vi "avalanche.vi"() -> ()   [LabVIEW 2018]
panel:
  out "Collision":bool
  out "High Score":u32
  in  "Difficulty":dbl
  out "Key Down":bool
  out "Key Up":bool
  out "Height":i32
  out "Key Right":bool
  out "Key Left":bool
  out "Final Score":i32
  out "% Passed":dbl
  in  "stop":bool
  out "Current Score":i32
  out "XY Graph":cluster{dbl[], i32[]}(graph)
  out "Position":dbl
  out "error out":errorcluster
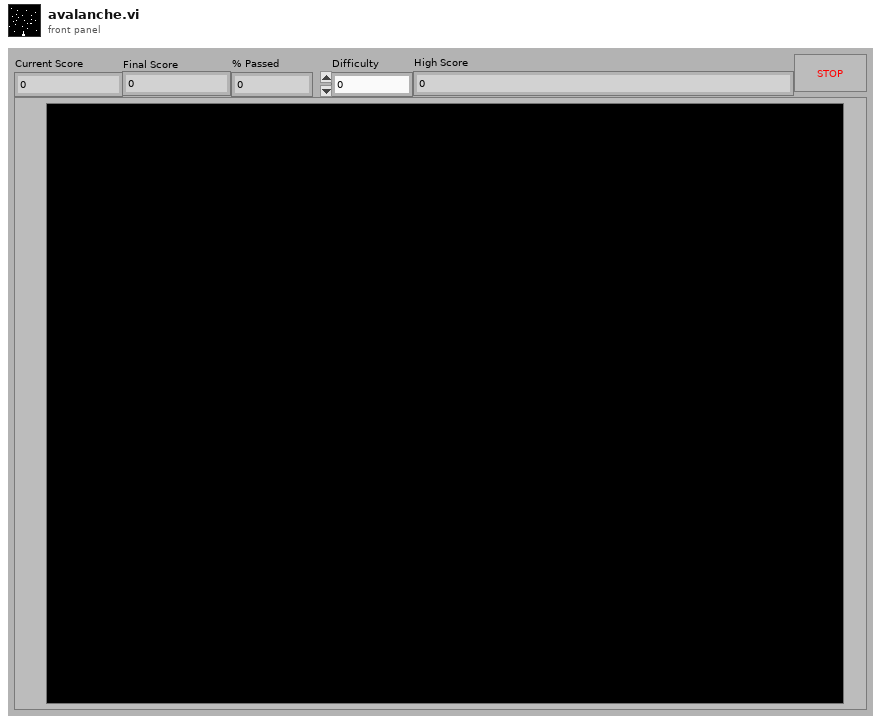
[diagram p1: front panel]
types:
  T1 = typedef "eventvkey.ctl" = enum16{"ASCII", "Enter", "Return", "Shift", "Ctrl", "Alt", "Cmd", "Opt", "Caps", "NumLock", "Clear", "Break", "Up", "Down", "Left", "Right", "Insert", "Delete", "Home", "End", "PageUp", "PageDown", "Escape", "Help", "Pause", "ScrollLock", "F1", "F2", "F3", "F4", "F5", "F6", "F7", "F8", "F9", "F10", "F11", "F12", "F13", "F14", "F15", "F16", "F17", "F18", "F19", "F20", "F21", "F22", "F23", "F24", "Play", "VolumeUp", "VolumeDown", "Mute", "Two Byte Char"}
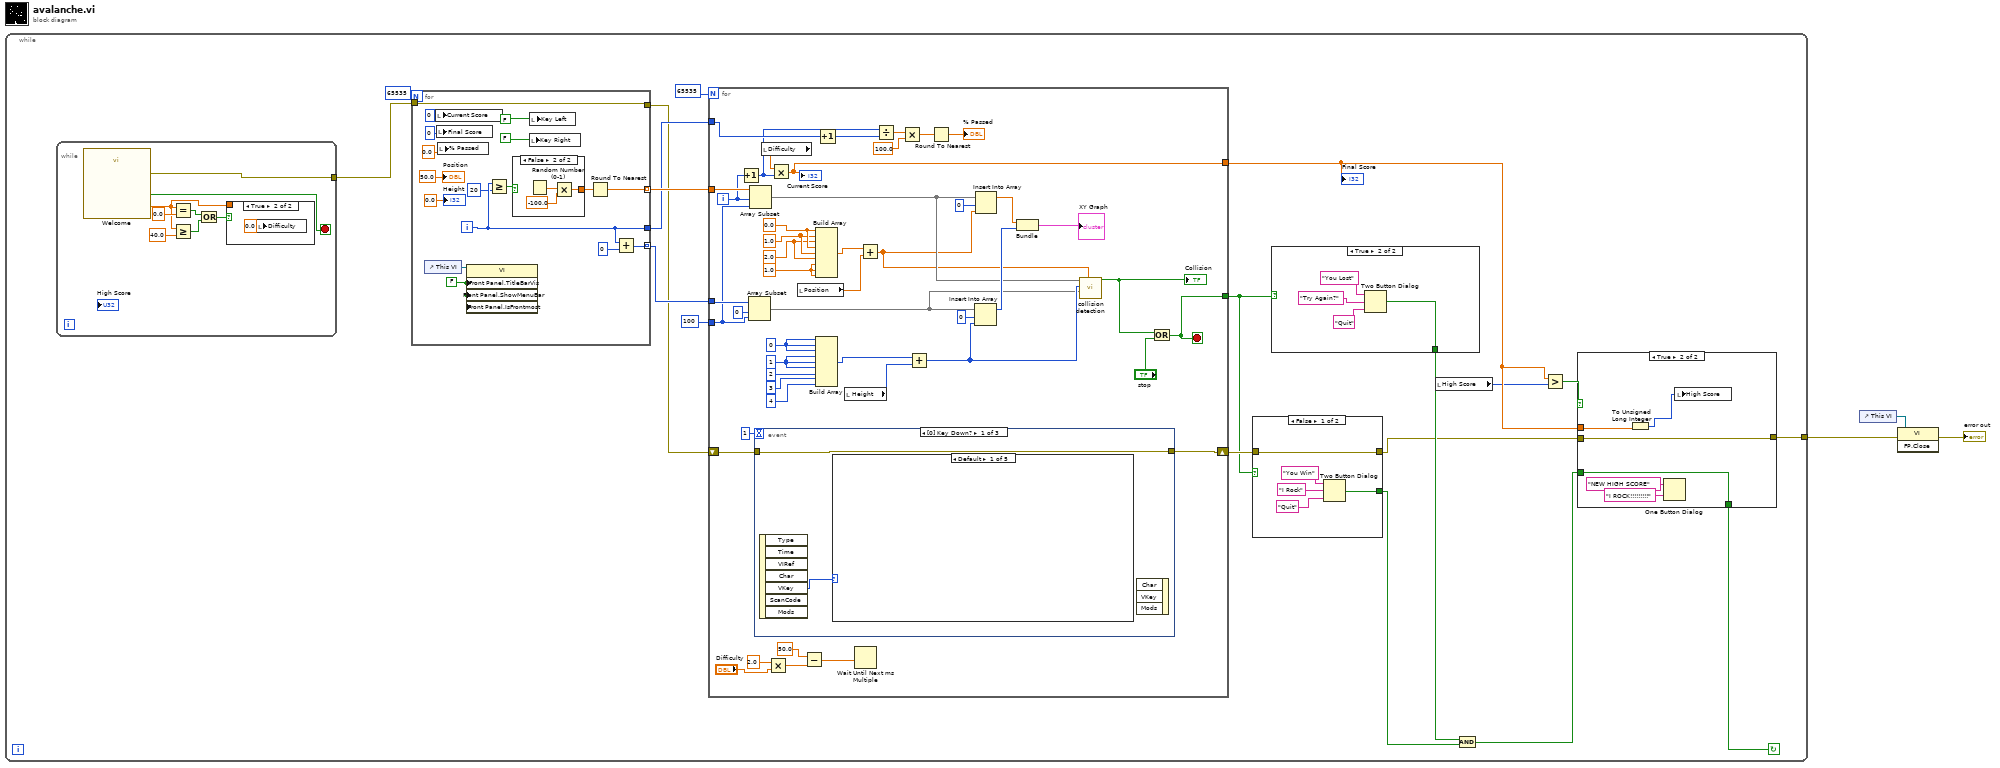
[diagram p0: block diagram]
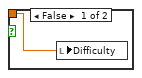
[diagram p3: hidden frame]
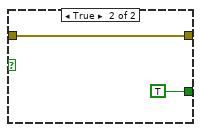
[diagram p4: hidden frame]
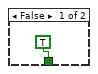
[diagram p5: hidden frame]
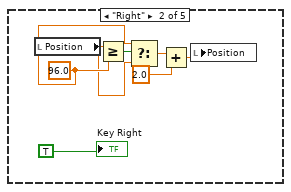
[diagram p6: hidden frame]
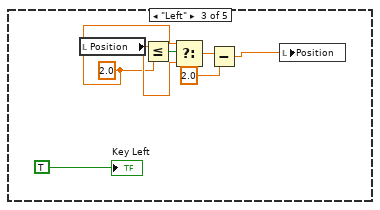
[diagram p7: hidden frame]
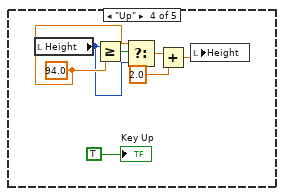
[diagram p8: hidden frame]
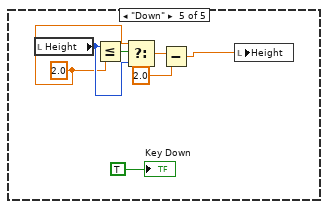
[diagram p9: hidden frame]
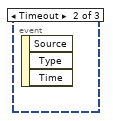
[diagram p10: hidden frame]
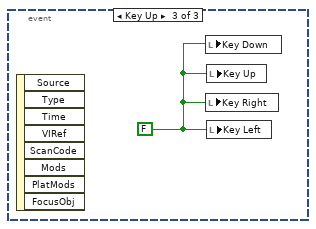
[diagram p11: hidden frame]
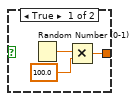
[diagram p12: hidden frame]
diagram:
  n1 = while {
    tunnel: [w8] -> w2
    stop <- w6 continue-if-true
    n2 = while {
      tunnel: [w37] -> w11
      stop <- w38 stop-if-true
      n3 = call "Welcome"() -> ("Difficulty 1-40"=w34:dbl, "OK"=w38:bool, "error out"=w37:errorcluster)  [unwired: 2 in, 15 out]
      n4 = Equal?(x=w34, y=0.0) -> (x = y?=w31:bool)
      n5 = Greater Or Equal?(x=w34, y=40.0) -> (x >= y?=w32:bool)
      n6 = Or(x=w31, y=w32) -> (x .or. y?=w35:bool)
      n7 = case shown="True" w35 {
        tunnel: w34 -> [w39 _]
        frame False {
          n8 = local write "Difficulty"(w39) -> ()
        }
        frame True {
          n9 = local write "Difficulty"(0.0 ("Difficulty")) -> ()
        }
      }
    }
    n10 = for {
      N: 65535 -> [_]
      tunnel: [w138] -> w21 mode=indexing
      tunnel: [w134] -> w17
      tunnel: w11 -> [w146]
      tunnel: [w146] -> w16
      tunnel: [w137] -> w19 mode=indexing
      i -> [w134]
      w131 = FALSE ("Front Panel Window:Title Bar Visible")
      n11 = control-ref of="This VI"() -> (w132:refnum<vi>)
      n12 = local write "Current Score"(0 ("Current Score")) -> ()
      n13 = local write "Final Score"(0 ("Final Score")) -> ()
      n14 = local write "% Passed"(0.0 ("% Passed")) -> ()
      n15 = property class="VI"(reference=w132, "Front Panel.TitleBarVis"=w131, "Front Panel.ShowMenuBar"=w131, "Front Panel.IsFrontmost"=w131) -> ()  [unwired: 1 in, 2 out]
      n16 = Greater Or Equal?(x=w134, y=20) -> (x >= y?=w135:bool)
      n17 = case shown="False" w135 {
        tunnel: [w148 w151] -> w147
        frame True {
          n18 = Random Number (0-1)() -> (number: 0 to 1=w150:dbl)
          n19 = Multiply(x=w150, y=100.0) -> (x*y=w148:dbl)
        }
        frame False {
          n20 = Random Number (0-1)() -> (number: 0 to 1=w153:dbl)
          n21 = Multiply(x=w153, y=-100.0) -> (x*y=w151:dbl)
        }
      }
      n22 = local write "Key Right"(FALSE ("Key Down")) -> ()
      n23 = local write "Key Left"(FALSE ("Key Up")) -> ()
      n24 = Round To Nearest(number=w147) -> (nearest integer value=w138:dbl)
      n25 = Add(x=w134, y=0) -> (x+y=w137:i32)
      "Position" <- 50.0 ("Position")
      "Height" <- 0.0 ("Height")
    }
    n26 = for {
      N: 65535 -> [_]
      tunnel: w21 -> [w98]
      tunnel: w19 -> [w99]
      tunnel: 100 -> [w97]
      tunnel: w17 -> [w58]
      tunnel: [w94] -> w14
      shift-right: [w70] -> w15
      shift-left: w16 -> [w69]
      tunnel: [w53] -> w5
      i -> [w95]
      stop <- w94 stop-if-true
      w86 = 1 ("element")
      w82 = 1.0 ("element")
      w87 = 0
      w79 = 2.0 ("new element/subarray")
      w81 = 0.0 ("new element/subarray")
      w80 = 1.0 ("new element/subarray")
      n27 = Increment(x=w95) -> (x+1=w57:i32)
      n28 = Array Subset(array=w99, index=0, length=w97) -> (w73:i32[])
      n29 = Array Subset(array=w98, index=w95, length=w97) -> (w72:dbl[])
      n30 = event shown="[0] Key Down?" {
        selector: _ -> [_ _ _]
        dyn-events: _ -> [_ _ _]
        timeout: 1 -> [_ _ _]
        tunnel: [w100 _ _] -> w70
        tunnel: w69 -> [w100 _ _]
        event Key Down? {
          n31 = event-data() -> ("VKey"=w101:T1)  [unwired: 7 out]
          n32 = case shown="Default" w101 {
            frame Default {
            }
            frame "Right" {
              w108 = 96.0 ("y")
              n33 = local read "Position"() -> (w107:dbl)
              n34 = Greater Or Equal?(x=w107, y=w108) -> (x >= y?=w106:bool)
              n35 = Select(t=w108, s=w106, f=w107) -> (s? t:f=w104:dbl)
              n36 = Add(x=w104, y=2.0) -> (x+y=w105:dbl)
              n37 = local write "Position"(w105) -> ()
              "Key Right" <- TRUE ("Key Up")
            }
            frame "Left" {
              w113 = 2.0 ("y")
              n38 = local read "Position"() -> (w114:dbl)
              n39 = Less Or Equal?(x=w114, y=w113) -> (x <= y?=w115:bool)
              n40 = Select(t=w113, s=w115, f=w114) -> (s? t:f=w111:dbl)
              n41 = Subtract(x=w111, y=2.0) -> (x-y=w110:dbl)
              n42 = local write "Position"(w110) -> ()
              "Key Left" <- TRUE ("Key Down")
            }
            frame "Up" {
              w121 = 94.0 ("y")
              n43 = local read "Height"() -> (w120:i32)
              n44 = Greater Or Equal?(x=w120, y=w121) -> (x >= y?=w119:bool)
              n45 = Select(t=w121, s=w119, f=w120) -> (s? t:f=w117:dbl)
              n46 = Add(x=w117, y=2.0) -> (x+y=w118:dbl)
              n47 = local write "Height"(w118) -> ()
              "Key Up" <- TRUE ("Key Up")
            }
            frame "Down" {
              w126 = 2.0 ("y")
              n48 = local read "Height"() -> (w127:i32)
              n49 = Less Or Equal?(x=w127, y=w126) -> (x <= y?=w128:bool)
              n50 = Select(t=w126, s=w128, f=w127) -> (s? t:f=w124:dbl)
              n51 = Subtract(x=w124, y=2.0) -> (x-y=w123:dbl)
              n52 = local write "Height"(w123) -> ()
              "Key Down" <- TRUE ("Key Down")
            }
          }
          n53 = event-data() -> ()  [unwired: 1 in, 4 out]
        }
        event Timeout {
          n54 = event-data() -> ()  [unwired: 4 out]
        }
        event Key Up {
          w130 = FALSE ("Key Down")
          n55 = event-data() -> ()  [unwired: 9 out]
          n56 = local write "Key Down"(w130) -> ()
          n57 = local write "Key Right"(w130) -> ()
          n58 = local write "Key Up"(w130) -> ()
          n59 = local write "Key Left"(w130) -> ()
        }
      }
      n60 = local read "Difficulty"() -> (w54:dbl)
      n61 = Multiply(x=2.0, y="Difficulty") -> (x*y=w65:dbl)
      n62 = Multiply(x=w54, y=w57) -> (x*y=w53:dbl)
      "Current Score" <- w53
      n63 = local read "Position"() -> (w77:dbl)
      n64 = Subtract(x=50.0 ("y"), y=w65) -> (x-y=w63:dbl)
      n65 = Build Array(w81, w80, w79, w81, w80, w79, w82, w82, w82) -> (w78:dbl[])
      n66 = Build Array(w87, w87, w87, w86, w86, w86, 2 ("element"), 3 ("element"), 4 ("element")) -> (w76:i32[])
      n67 = Increment(x=w58) -> (x+1=w59:i32)
      n68 = local read "Height"() -> (w75:i32)
      n69 = Wait Until Next ms Multiple(millisecond multiple=w63) -> ()  [unwired: 1 out]
      n70 = Add(x=w78, y=w77) -> (x+y=w71:dbl[])
      n71 = Divide(x=w57, y=w59) -> (x/y=w62:dbl)
      n72 = Multiply(x=w62, y=100.0) -> (x*y=w61:dbl)
      n73 = Add(x=w76, y=w75) -> (x+y=w74:i32[])
      n74 = Round To Nearest(number=w61) -> (nearest integer value=→"% Passed":dbl)
      n75 = Insert Into Array(array=w73, index=0, new element=w74) -> (w89:i32[])
      n76 = Insert Into Array(array=w72, index=0, new element=w71) -> (w90:dbl[])
      n77 = Bundle(w90, w89) -> (→"XY Graph":cluster{dbl[], i32[]})  [unwired: 1 out]
      n78 = call "collision detection.vi"("y values 2"=w71, "x values"=w73, "x values 2"=w74, "y values"=w72) -> ("Collision"=w55:bool)  [unwired: 1 in, 6 out]
      "Collision" <- w55
      n79 = Or(x=w55, y="stop") -> (x .or. y?=w94:bool)
    }
    "Final Score" <- w5
    n80 = case shown="False" w14 {
      tunnel: w15 -> [w44 w47]
      tunnel: [w44 w47] -> w9
      tunnel: [w41 TRUE ("T button?")] -> w12
      frame False {
        n81 = Two Button Dialog(message="You Win", 1:"Quit" ("F button name (\"Cancel\")"), 2:"I Rock" ("button name (\"OK\")")) -> (T button?=w41:bool)
      }
      frame True {
      }
    }
    n82 = case shown="True" w14 {
      tunnel: [TRUE ("T button?") w49] -> w13
      frame False {
      }
      frame True {
        n83 = Two Button Dialog(message="You Lost", 1:"Quit" ("F button name (\"Cancel\")"), 2:"Try Again?" ("button name (\"OK\")")) -> (T button?=w49:bool)
      }
    }
    n84 = local read "High Score"() -> (w4:u32)
    n85 = And(x=w13, y=w12) -> (x .and. y?=w7:bool)
    n86 = Greater?(x=w5, y=w4) -> (0:w10:bool)
    n87 = case shown="True" w10 {
      tunnel: w9 -> [w23 w26]
      tunnel: w5 -> [_ w28]
      tunnel: [w23 w26] -> w8
      tunnel: w7 -> [w24 w27]
      tunnel: [w24 w27] -> w6
      frame False {
      }
      frame True {
        n88 = To Unsigned Long Integer(number=w28) -> (unsigned 32bit integer=w25:u32)
        n89 = One Button Dialog(message="NEW HIGH SCORE", button name ("OK")="I ROCK!!!!!!!!!") -> ()  [unwired: 1 out]
        n90 = local write "High Score"(w25) -> ()
      }
    }
  }
  n91 = control-ref of="This VI"() -> (w1:refnum<vi>)
  n92 = invoke class="VI" method="FP.Close"(reference=w1, error in=w2) -> (error out=→"error out":errorcluster)  [unwired: 1 in, 2 out]
